vi "csb can deserialize.vi"(0 "payload":u8[](array[numeric]), 1 "len":i32, 2 "t_dev":dbl[](array[numeric]), 3 "id":u32[](array[numeric]), 4 "flags":u16[](array[numeric]), 5 "dlc":u8[](array[numeric]), 6 "data_len":u8[](array[numeric]), 7 "error in (no error)":errorcluster, 9 "max_frames":i32, 11 "data":u8[](array[numeric])) -> (18 "data out":u8[](array[numeric]), 19 "function return":i32, 20 "n_frames":i32, 21 "decode_errors":i32, 22 "t_dev out":dbl[](array[numeric]), 23 "id out":u32[](array[numeric]), 24 "flags out":u16[](array[numeric]), 25 "dlc out":u8[](array[numeric]), 26 "data_len out":u8[](array[numeric]), 27 "error out":errorcluster)   [LabVIEW 2021, in "CANsub_Codec.lvlib"]
doc: "int32_t csb_can_deserialize(const uint8_t *payload, int32_t len,\n double *t_dev, uint32_t *id, uint16_t *flags, uint8_t *dlc,\n uint8_t *data_len, uint8_t *data, int32_t max_frames,\n int32_t *n_frames, int32_t *decode_errors);"
uses:
  CANsub_Codec.lvlib
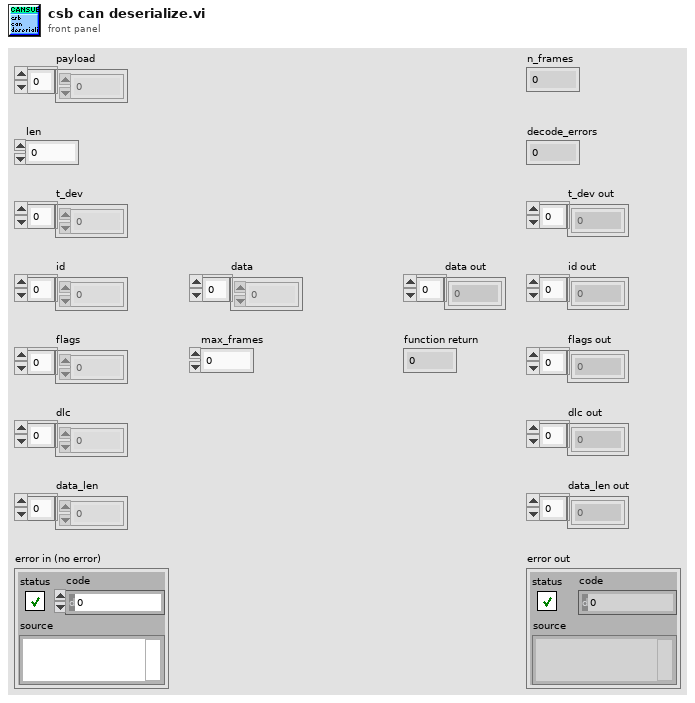
[diagram p1: front panel]
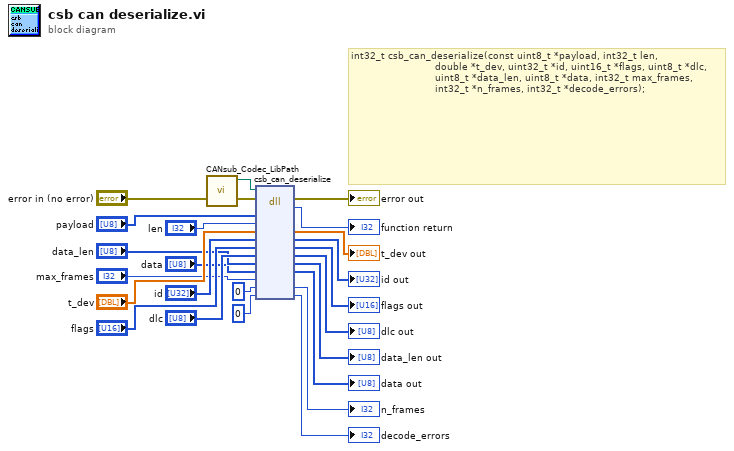
[diagram p0: block diagram]
diagram:
  # "int32_t csb_can_deserialize(const uint8_t *payload, int32_t len,\n                            double *t_dev, uint32_t *id, uint16_t *flags, uint8_t *dlc,\n                            uint8_t *data_len, uint8_t *data, int32_t max_frames,\n                            int32_t *n_frames, int32_t *decode_errors);"
  n1 = call "CANsub_Codec_LibPath.vi"() -> ("Path"=w1:path)  [unwired: 11 in]
  n2 = dll-call lib="libcansub_codec.*" fn="csb_can_deserialize"(path in=w1, error in="error in (no error)", "payload"="payload", "len"="len", "t_dev"="t_dev", "id"="id", "flags"="flags", "dlc"="dlc", "data_len"="data_len", "data"="data", "max_frames"="max_frames", "n_frames"=0, "decode_errors"=0) -> (error out=→"error out":errorcluster, "return type"=→"function return":i32, "t_dev"=→"t_dev out":dbl[], "id"=→"id out":u32[], "flags"=→"flags out":u16[], "dlc"=→"dlc out":u8[], "data_len"=→"data_len out":u8[], "data"=→"data out":u8[], "n_frames"=→"n_frames":i32, "decode_errors"=→"decode_errors":i32)  [unwired: 4 in, 1 out]
